vi "work2_cooker_draft_module.vi"() -> ()   [LabVIEW 2026]
panel:
  out "Notifications":string
  in  "Nb_Meals":dbl
  in  "Nb_Burgers":dbl
  in  "Cook Burgers":bool
  in  "Cook Meal":bool
  in  "Stop":bool
  out "CookedBurgers":i32
  out "CookedMeal":i32
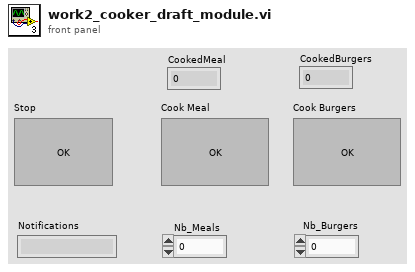
[diagram p1: front panel]
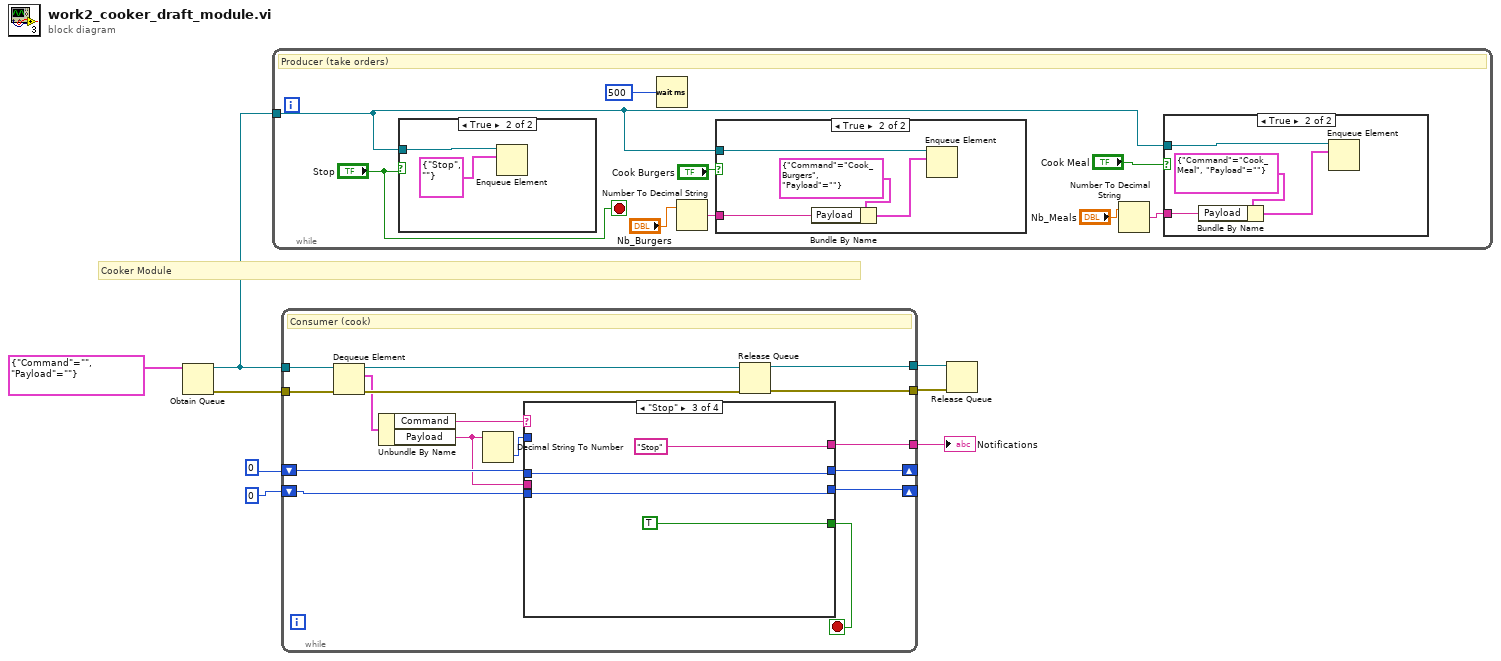
[diagram p0: block diagram]
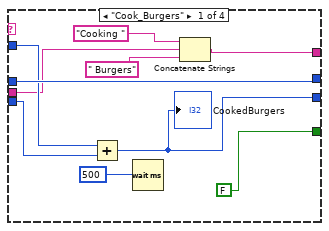
[diagram p2: hidden frame]
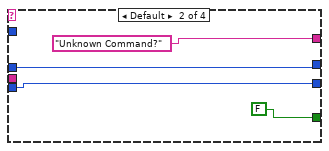
[diagram p3: hidden frame]
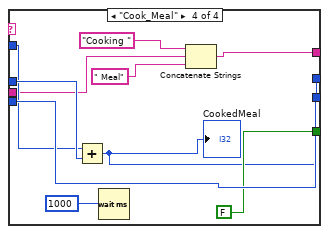
[diagram p4: hidden frame]
diagram:
  # "Cooker Module"
  n1 = Obtain Queue(element data type=cluster{"Command":string, "Payload":string} {"Command"="", "Payload"=""} ("Orders")) -> (queue out=w8:refnum<queue>, error out=w7:errorcluster)  [unwired: 4 in, 1 out]
  n2 = while {
    tunnel: w8 -> [w15]
    stop <- "Stop" stop-if-true
    # "Producer (take orders)"
    n3 = case shown="True" "Stop" {
      tunnel: w15 -> [_ w27]
      frame False {
      }
      frame True {
        n4 = Enqueue Element(queue=w27, element=cluster{"Stop":string, string} {"Stop"="Stop", ""} ("Orders")) -> ()  [unwired: 2 in, 3 out]
      }
    }
    n5 = Wait (ms)(milliseconds to wait=500) -> ()  [unwired: 1 out]
    n6 = Number To Decimal String(number="Nb_Burgers") -> (decimal integer string=w13:string)  [unwired: 1 in]
    n7 = case shown="True" "Cook Burgers" {
      tunnel: w15 -> [_ w25]
      tunnel: w13 -> [_ w22]
      frame False {
      }
      frame True {
        n8 = Bundle By Name(cluster=cluster{"Command":string, "Payload":string} {"Command"="Cook_Burgers", "Payload"=""} ("Orders"), "Payload"=w22) -> (w23:cluster{"Command":string, "Payload":string})
        n9 = Enqueue Element(queue=w25, element=w23) -> ()  [unwired: 2 in, 3 out]
      }
    }
    n10 = Number To Decimal String(number="Nb_Meals") -> (decimal integer string=w9:string)  [unwired: 1 in]
    n11 = case shown="True" "Cook Meal" {
      tunnel: w15 -> [_ w21]
      tunnel: w9 -> [_ w20]
      frame False {
      }
      frame True {
        n12 = Bundle By Name(cluster=cluster{"Command":string, "Payload":string} {"Command"="Cook_Meal", "Payload"=""} ("Orders"), "Payload"=w20) -> (w18:cluster{"Command":string, "Payload":string})
        n13 = Enqueue Element(queue=w21, element=w18) -> ()  [unwired: 2 in, 3 out]
      }
    }
  }
  n14 = while {
    tunnel: w8 -> [w41]
    tunnel: w7 -> [w40]
    tunnel: [w39] -> w2
    tunnel: [w38] -> w5
    shift-right: [w34] -> _
    shift-left: 0 -> [w35]
    shift-right: [w32] -> _
    shift-left: 0 -> [w33]
    tunnel: [w29] -> w1
    stop <- w36 stop-if-true
    # "Consumer (cook)"
    n15 = Dequeue Element(queue=w41, error in (no error)=w40) -> (queue out=w38:refnum<queue>, element=w37:cluster{"Command":string, "Payload":string}, error out=w39:errorcluster)  [unwired: 1 in, 1 out]
    n16 = Unbundle By Name(w37) -> ("Command"=w30:string, "Payload"=w28:string)
    n17 = Decimal String To Number(string=w28) -> (number=w31:i32)  [unwired: 2 in, 1 out]
    n18 = case shown="\"Stop\"" w30 {
      tunnel: [FALSE FALSE TRUE FALSE] -> w36
      tunnel: w31 -> [w46 _ _ w64]
      tunnel: w35 -> [w50 w55 w58 w66]
      tunnel: [w50 w55 w58 w65] -> w34
      tunnel: w33 -> [w48 w54 w57 w68]
      tunnel: [w47 w54 w57 w68] -> w32
      tunnel: [w43 "Unknown Command?" "Stop" w63] -> w29
      tunnel: w28 -> [w42 _ _ w61]
      frame "Cook_Burgers" {
        n19 = Add(x=w46, y=w48) -> (x+y=w47:i32)
        "CookedBurgers" <- w47
        n20 = Wait (ms)(milliseconds to wait=500) -> ()  [unwired: 1 out]
        n21 = Concatenate Strings("Cooking ", w42, " Burgers") -> (w43:string)
      }
      frame Default {
      }
      frame "Stop" {
      }
      frame "Cook_Meal" {
        n22 = Add(x=w64, y=w66) -> (x+y=w65:i32)
        "CookedMeal" <- w65
        n23 = Wait (ms)(milliseconds to wait=1000) -> ()  [unwired: 1 out]
        n24 = Concatenate Strings("Cooking ", w61, " Meal") -> (w63:string)
      }
    }
  }
  "Notifications" <- w1
  n25 = Release Queue(queue=w5, error in (no error)=w2) -> ()  [unwired: 1 in, 3 out]
  n26 = Release Queue(queue=w5, error in (no error)=w2) -> ()  [unwired: 1 in, 3 out]
